vi "PLC_WriteWord.vi"(8 "error in (no error)":errorcluster, 9 "Value":u16, 10 "Address D":u16, 11 "PLC Conn":refnum<visa-resource-name>) -> (0 "error out":errorcluster, 3 "PLC Conn out":refnum<visa-resource-name>)   [LabVIEW 2018]
doc: "Use this template to build a VI to use as a subVI."
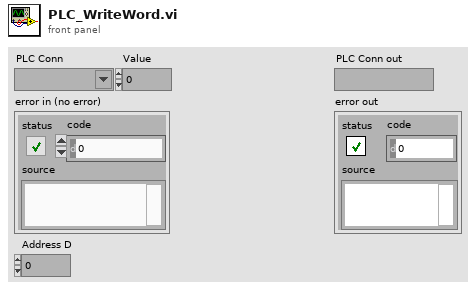
[diagram p1: front panel]
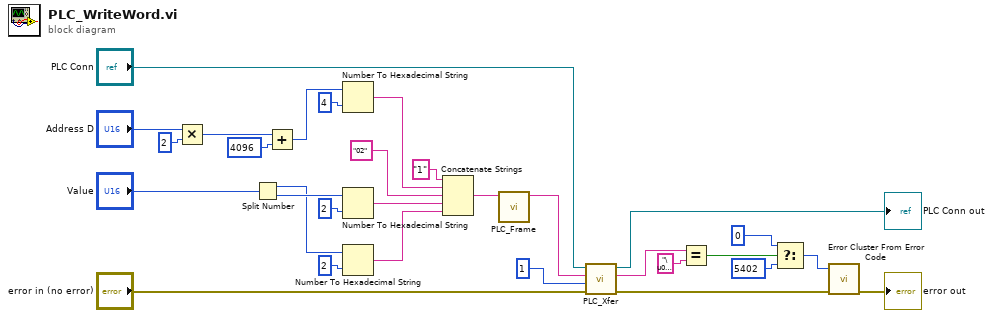
[diagram p0: block diagram]
diagram:
  n1 = Multiply(x="Address D", y=u16 2) -> (x*y=w27:u16)
  n2 = Split Number(x="Value") -> (hi(x)=w21:u8, lo(x)=w23:u8)
  n3 = Add(x=w27, y=u16 4096) -> (x+y=w25:u16)
  n4 = Number To Hexadecimal String(1:i16 4 ("width (-)"), 2:w25) -> (0:w18:string)
  n5 = Number To Hexadecimal String(1:i16 2 ("width (-)"), 2:w23) -> (0:w16:string)
  n6 = Number To Hexadecimal String(1:i16 2 ("width (-)"), 2:w21) -> (0:w15:string)
  n7 = Concatenate Strings("1", w18, "02", w16, w15) -> (w14:string)
  n8 = call "PLC_Frame.vi"("Payload"=w14) -> ("Frame"=w13:string)  [unwired: 10 in]
  n9 = call "PLC_Xfer.vi"("error in (no error)"="error in (no error)", "RX Bytes"=u32 1, "TX"=w13, "PLC Conn"="PLC Conn") -> ("error out"=w3:errorcluster, "RX"=w9:string, "PLC Conn out"=→"PLC Conn out":refnum<visa-resource-name>)  [unwired: 5 in]
  n10 = Equal?(x=w9, y="\u0006") -> (x = y?=w7:bool)
  n11 = Select(t=0, s=w7, f=5402) -> (s? t:f=w4:i32)
  n12 = call <vilib>:"Error Cluster From Error Code.vi"("error in (no error)"=w3, "error code (0)"=w4) -> ("error out"=→"error out":errorcluster)  [unwired: 7 in]
